vi "Update Layout.vi"(8 "error in (no error)":errorcluster, 10 "UI Refs":T1, 11 "ArrayManager in":refnum<class "ArrayManager.lvclass">) -> (0 "error out":errorcluster, 3 "ArrayManager out":refnum<class "ArrayManager.lvclass">)   [LabVIEW 2020, in "OOPanel.lvlib" / "ArrayManager.lvclass"]
uses:
  ArrayManager.lvclass
  UI Refs.ctl
  ArrayManager.lvclass/ArrayManager.ctl
  ArrayPanel/ArrayPanel.lvclass
  C:/dev/LabVIEW/lv-oopanel/OOPanel/Panel/Panel.lvclass
  Manager/Manager.lvclass
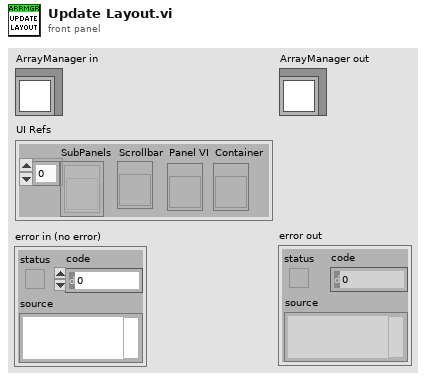
[diagram p1: front panel]
types:
  T1 = typedef "OOPanel.lvlib/ArrayManager.lvclass/UI Refs.ctl" = cluster{"SubPanels":refnum<vi>[], "Scrollbar":refnum<vi>, "Panel VI":refnum<vi>, "Container":refnum<vi>}
  T2 = typedef "OOPanel.lvlib/ArrayPanel.lvclass/Desired Size.ctl" = cluster{"Width":u32, "Height":u32}
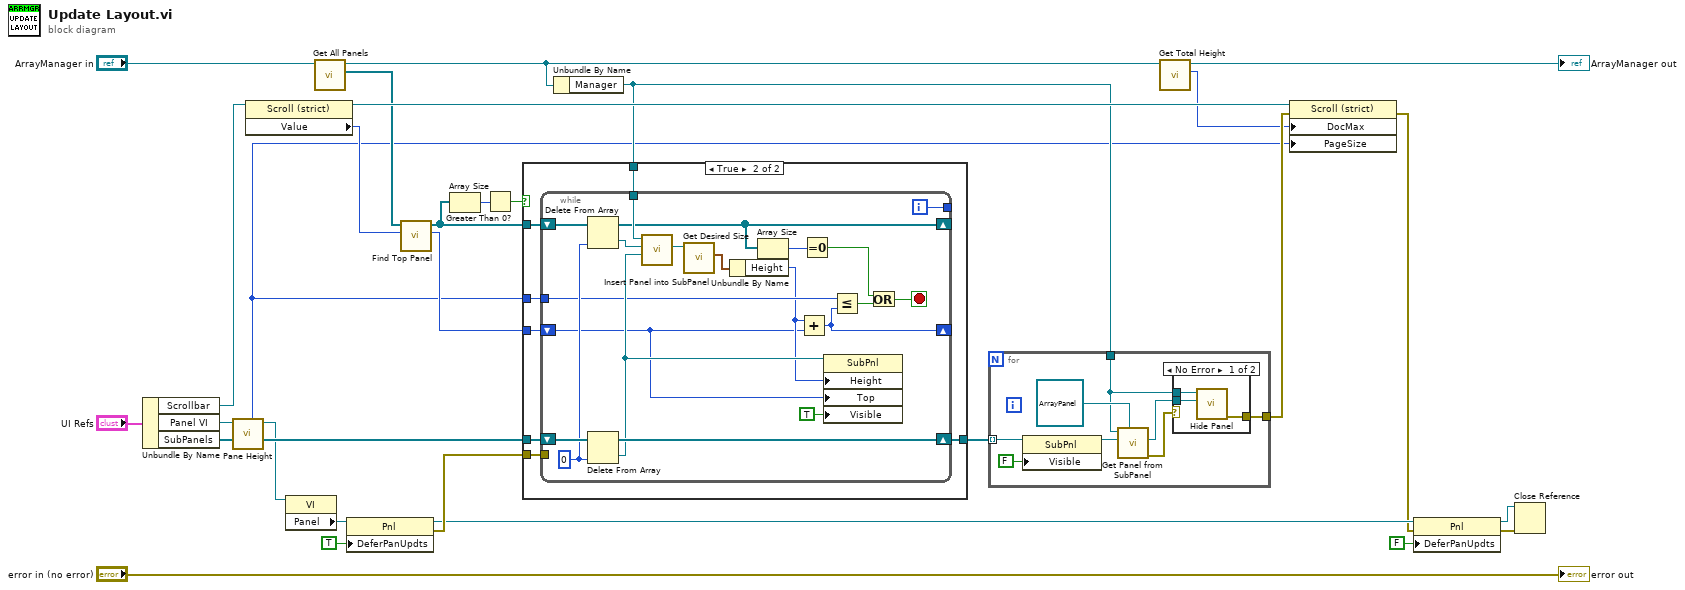
[diagram p0: block diagram]
diagram:
  n1 = Unbundle By Name("UI Refs") -> ("Scrollbar"=w26:refnum<vi>, "Panel VI"=w23:refnum<vi>, "SubPanels"=w24:refnum<vi>[])
  n2 = call "Pane Height.vi"("Panel VI in"=w23) -> ("Panel VI"=w22:refnum<vi>, "Height"=w4:u32)  [unwired: 9 in]
  n3 = property class="Scroll (strict)"(reference=w26) -> (reference out=w25:refnum<vi>, "Value"=w6:i32)  [unwired: 1 in, 1 out]
  n4 = property class="VI"(reference=w22) -> ("Panel"=w21:refnum<vi>)  [unwired: 1 in, 2 out]
  n5 = call "Get All Panels.vi"("PanelArray in"="ArrayManager in") -> ("Panels"=w7:refnum<class "ArrayPanel.lvclass">[], "PanelArray out"=w10:refnum<class "ArrayManager.lvclass">)  [unwired: 8 in, 1 out]
  n6 = property class="Pnl"(reference=w21, "DeferPanUpdts"=TRUE ("Defer Panel Updates")) -> (reference out=w17:refnum<vi>, error out=w19:errorcluster)  [unwired: 1 in]
  n7 = call "Find Top Panel.vi"("Scroll"=w6, "All Panels"=w7) -> ("Start"=w5:i32, "Panels"=w3:refnum<class "ArrayPanel.lvclass">[])  [unwired: 8 in]
  n8 = Array Size(array=w3) -> (size(s)=w2:i32)
  n9 = Greater Than 0?(x=w2) -> (x > 0?=w1:bool)
  n10 = Unbundle By Name(w10) -> ("Manager"=w11:refnum<class "Manager.lvclass">)
  n11 = case shown="True" w1 {
    tunnel: w24 -> [w30 w37]
    tunnel: w19 -> [_ w36]
    tunnel: [w30 w35] -> w12
    tunnel: w11 -> [_ w34]
    tunnel: w5 -> [_ w33]
    tunnel: w4 -> [_ w32]
    tunnel: w3 -> [_ w31]
    frame False {
    }
    frame True {
      n12 = while {
        shift-right: [w56] -> w35
        shift-left: w37 -> [w57]
        tunnel: w32 -> [w47]
        tunnel: w36 -> [_]
        shift-right: [w43] -> _
        shift-left: w31 -> [w55]
        tunnel: w34 -> [w53]
        shift-right: [w46] -> _
        shift-left: w33 -> [w38]
        tunnel: [w44] -> _
        i -> [w44]
        stop <- w41 stop-if-true
        w54 = 0 ("index")
        n13 = Delete From Array(array=w55, index=w54) -> (deleted portion=w52:refnum<class "ArrayPanel.lvclass">, array with subset deleted=w43:refnum<class "ArrayPanel.lvclass">[])  [unwired: 1 in]
        n14 = Delete From Array(array=w57, index=w54) -> (deleted portion=w51:refnum<vi>, array with subset deleted=w56:refnum<vi>[])  [unwired: 1 in]
        n15 = call "Insert Panel into SubPanel.vi"("SubPanel"=w51, "Panel In"=w52, "Manager in"=w53) -> ("Panel"=w49:refnum<class "ArrayPanel.lvclass">)  [unwired: 6 in, 2 out]
        n16 = call-dynamic "Get Desired Size.vi"("ArrayPanel in"=w49) -> ("Desired Size"=w48:T2)  [unwired: 8 in, 2 out]
        n17 = Unbundle By Name(w48) -> ("Height"=w39:u32)
        n18 = Array Size(array=w43) -> (size(s)=w42:i32)
        n19 = Add(x=w39, y=w38) -> (x+y=w46:u32)
        n20 = Equal To 0?(x=w42) -> (x = 0?=w40:bool)
        n21 = property class="SubPnl"(reference=w51, "Height"=w39, "Top"=w38, "Visible"=TRUE) -> ()  [unwired: 1 in, 2 out]
        n22 = Less Or Equal?(x=w47, y=w46) -> (x <= y?=w45:bool)
        n23 = Or(x=w40, y=w45) -> (x .or. y?=w41:bool)
      }
    }
  }
  n24 = for {
    tunnel: w12 -> [w61] mode=indexing
    tunnel: w11 -> [w62]
    tunnel: [w58] -> w29
    n25 = property class="SubPnl"(reference=w61, "Visible"=FALSE) -> (reference out=w60:refnum<vi>)  [unwired: 1 in, 1 out]
    n26 = call "Get Panel from SubPanel.vi"("Panel Type (Panel)"=refnum<class "ArrayPanel.lvclass"> refnum ("OOPanel.lvlib:ArrayPanel.lvclass"), "SubPanel"=w60, "Manager in"=w62) -> ("error out"=w64:errorcluster, "Panel"=w63:refnum<class "ArrayPanel.lvclass">)  [unwired: 6 in, 1 out]
    n27 = case shown="No Error" w64 {
      tunnel: w63 -> [w68 _]
      tunnel: w62 -> [w67 _]
      tunnel: [w66 _] -> w58
      frame No Error {
        n28 = call "Hide Panel.vi"("Panel In"=w68, "Manager in"=w67) -> ("error out"=w66:errorcluster)  [unwired: 7 in, 2 out]
      }
      frame Error {
      }
    }
  }
  n29 = call "Get Total Height.vi"("ArrayManager in"=w10) -> ("Total Height"=w8:u32, "ArrayManager out"=→"ArrayManager out":refnum<class "ArrayManager.lvclass">)  [unwired: 8 in, 1 out]
  n30 = property class="Scroll (strict)"(reference=w25, error in=w29, "DocMax"=w8, "PageSize"=w4) -> (error out=w15:errorcluster)  [unwired: 1 out]
  n31 = property class="Pnl"(reference=w17, error in=w15, "DeferPanUpdts"=FALSE ("Defer Panel Updates")) -> (reference out=w13:refnum<vi>, error out=w14:errorcluster)
  n32 = Close Reference(reference=w13, error in (no error)=w14) -> ()  [unwired: 1 out]
  "error out" <- "error in (no error)"
